vi "Host - Refresh All.vi"(8 "error in (no error)":errorcluster, 10 "ignore errors (T)":bool=TRUE, 11 "serverName":string="10.0.18.244") -> (0 "error out":errorcluster, 3 "serverName":string="10.0.18.244")   [LabVIEW 2020, in "SEECD System Explorer.lvlib"]
uses:
  SEECD System Explorer.lvlib
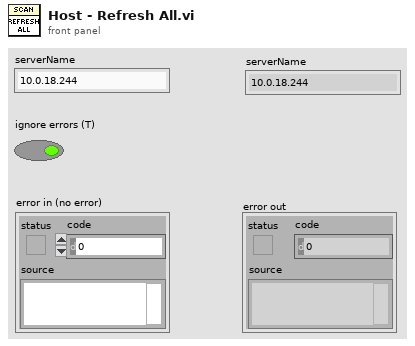
[diagram p1: front panel]
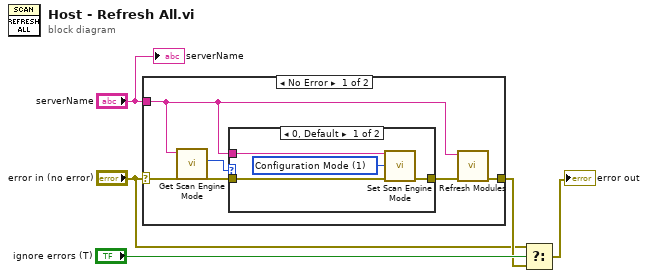
[diagram p0: block diagram]
diagram:
  n1 = case shown="No Error" "error in (no error)" {
    selector: "error in (no error)" -> [w9 w17]
    tunnel: "serverName" -> [w7 _]
    tunnel: [w6 w17] -> w3
    frame No Error {
      n2 = call <vilib>:"Get Scan Engine Mode.vi"("error in (no error)"=w9, "target address (localhost)"=w7) -> ("error out"=w11:errorcluster, "mode"=w10:i32)  [unwired: 8 in]
      n3 = case shown="0, Default" w10 {
        tunnel: w7 -> [w14 _]
        tunnel: w11 -> [w13 w16]
        tunnel: [w12 w16] -> w8
        frame 0, Default {
          w15 = 1 items=["Configuration Mode"=1, "Active Mode"=2] ("mode (Active Mode)")
          n4 = call <vilib>:"Set Scan Engine Mode.vi"("target address (localhost)"=w14, "mode (Active Mode)"=w15, "error in (no error)"=w13) -> ("error out"=w12:errorcluster)  [unwired: 12 in]
        }
        frame 1 {
        }
      }
      n5 = call <vilib>:"Refresh Modules.vi"("error in (no error)"=w8, "target address (localhost)"=w7) -> ("error out"=w6:errorcluster)  [unwired: 9 in]
    }
    frame Error {
    }
  }
  n6 = Select(t="error in (no error)", s="ignore errors (T)", f=w3) -> (s? t:f=→"error out":errorcluster)
  "serverName" <- "serverName"
